vi "Register gRPC Methods.vi"(8 "error in (no error)":errorcluster, 11 "gRPC service in":refnum<class "CanReaderCansub.lvclass">) -> (0 "error out":errorcluster, 3 "gRPC service out":refnum<class "CanReaderCansub.lvclass">)   [LabVIEW 2021, in "CanReaderCansub_server.lvlib" / "CanReaderCansub.lvclass"]
uses:
  CanReaderCansub.lvclass
  typeDefs/Server Internal UEs.ctl
  typeDefs/Server Internal Message.ctl
  typeDefs/Server gRPC UEs.ctl
  <vilib>/gRPC/LabVIEW gRPC Library/Server API/typeDefs/gRPCId Cluster.ctl
  <vilib>/gRPC/LabVIEW gRPC Library/Shared/grpcId.ctl
  CanReaderCansub.lvclass/CanReaderCansub.ctl
  <vilib>/gRPC/LabVIEW gRPC Library/grpc-lvsupport-release.lvlib
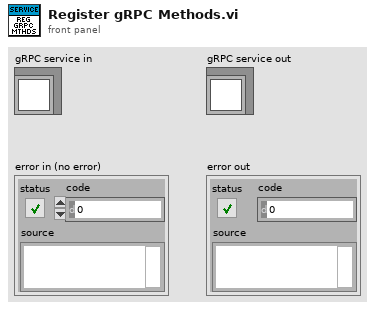
[diagram p1: front panel]
types:
  T1 = typedef "CanReaderCansub_server.lvlib/CanReaderCansub.lvclass/Server gRPC UEs.ctl" = cluster{"CanReaderCansub GetDevices gRPC UE":refnum<user-event>, "CanReaderCansub GetStatistics gRPC UE":refnum<user-event>, "CanReaderCansub SetInterfaceBlink gRPC UE":refnum<user-event>, "CanReaderCansub GetCANStatus gRPC UE":refnum<user-event>}
  T2 = typedef "CanReaderCansub_server.lvlib/CanReaderCansub.lvclass/Server Internal UEs.ctl" = cluster{"CanReaderCansub GetDevices Internal UE":refnum<user-event>, "CanReaderCansub GetStatistics Internal UE":refnum<user-event>, "CanReaderCansub SetInterfaceBlink Internal UE":refnum<user-event>, "CanReaderCansub GetCANStatus Internal UE":refnum<user-event>}
  T3 = typedef "grpc-lvsupport-release.lvlib/grpcId.ctl" = u64
  T4 = typedef "CanReaderCansub_server.lvlib/CanReaderCansub.lvclass/Server Internal Message UE.ctl" = refnum<user-event>
  T5 = typedef "grpc-lvsupport-release.lvlib/gRPCId Cluster UE.ctl" = refnum<user-event>
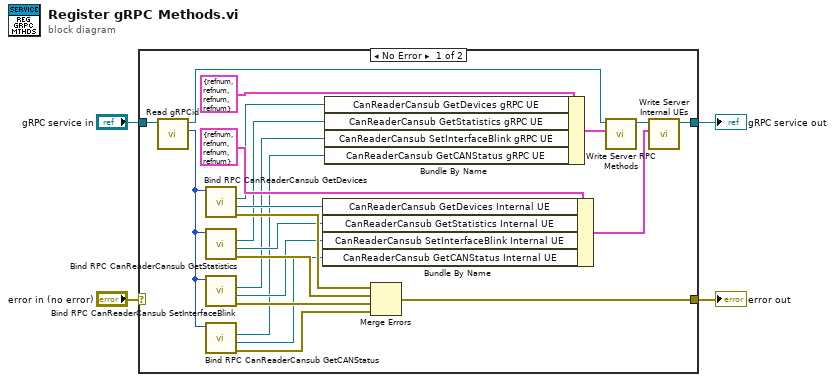
[diagram p0: block diagram]
diagram:
  n1 = case shown="No Error" "error in (no error)" {
    selector: "error in (no error)" -> [_ w27]
    tunnel: "gRPC service in" -> [w18 w28]
    tunnel: [w26 w27] -> w3
    tunnel: [w25 w28] -> w2
    frame No Error {
      n2 = call-dynamic "Read gRPCid.vi"("gRPC service in"=w18) -> ("gRPCid"=w17:T3, "gRPC service out"=w19:refnum<class "CanReaderCansub.lvclass">)  [unwired: 8 in, 1 out]
      n3 = call "Bind RPC CanReaderCansub GetDevices.vi"("gRPCid server in"=w17) -> ("error out"=w16:errorcluster, "CanReaderCansub GetDevices Internal UE"=w14:T4, "CanReaderCansub GetDevices gRPC UE"=w15:T5)  [unwired: 7 in, 1 out]
      n4 = call "Bind RPC CanReaderCansub GetStatistics.vi"("gRPCid server in"=w17) -> ("error out"=w13:errorcluster, "CanReaderCansub GetStatistics Internal UE"=w11:T4, "CanReaderCansub GetStatistics gRPC UE"=w12:T5)  [unwired: 7 in, 1 out]
      n5 = call "Bind RPC CanReaderCansub SetInterfaceBlink.vi"("gRPCid server in"=w17) -> ("error out"=w10:errorcluster, "CanReaderCansub SetInterfaceBlink Internal UE"=w8:T4, "CanReaderCansub SetInterfaceBlink gRPC UE"=w9:T5)  [unwired: 7 in, 1 out]
      n6 = call "Bind RPC CanReaderCansub GetCANStatus.vi"("gRPCid server in"=w17) -> ("error out"=w7:errorcluster, "CanReaderCansub GetCANStatus Internal UE"=w5:T4, "CanReaderCansub GetCANStatus gRPC UE"=w6:T5)  [unwired: 7 in, 1 out]
      n7 = Bundle By Name ("Bundle Internal UEs")(cluster=T2 {"CanReaderCansub GetDevices Internal UE"=refnum, "CanReaderCansub GetStatistics Internal UE"=refnum, "CanReaderCansub SetInterfaceBlink Internal UE"=refnum, "CanReaderCansub GetCANStatus Internal UE"=refnum} ("Server Internal UEs"), "CanReaderCansub GetDevices Internal UE"=w14, "CanReaderCansub GetStatistics Internal UE"=w11, "CanReaderCansub SetInterfaceBlink Internal UE"=w8, "CanReaderCansub GetCANStatus Internal UE"=w5) -> (w24:T2)
      n8 = Bundle By Name ("Bundle gRPC UEs")(cluster=T1 {"CanReaderCansub GetDevices gRPC UE"=refnum, "CanReaderCansub GetStatistics gRPC UE"=refnum, "CanReaderCansub SetInterfaceBlink gRPC UE"=refnum, "CanReaderCansub GetCANStatus gRPC UE"=refnum} ("gRPC Server Method Events"), "CanReaderCansub GetDevices gRPC UE"=w15, "CanReaderCansub GetStatistics gRPC UE"=w12, "CanReaderCansub SetInterfaceBlink gRPC UE"=w9, "CanReaderCansub GetCANStatus gRPC UE"=w6) -> (w21:T1)
      n9 = Merge Errors(w16, w13, w10, w7) -> (w26:errorcluster)
      n10 = call "Write Server RPC Methods.vi"("Server RPC Methods"=w21, "gRPC service in"=w19) -> ("gRPC service out"=w22:refnum<class "CanReaderCansub.lvclass">)  [unwired: 8 in, 1 out]
      n11 = call "Write Server Internal UEs.vi"("Server Internal UEs"=w24, "gRPC service in"=w22) -> ("gRPC service out"=w25:refnum<class "CanReaderCansub.lvclass">)  [unwired: 8 in, 1 out]
    }
    frame Error {
    }
  }
  "error out" <- w3
  "gRPC service out" <- w2
